vi "Select_Profile.vi"(0 "Enum":T1, 3 "error in":errorcluster) -> (7 "selected path":path, 10 "error out":errorcluster)   [LabVIEW 2021]
uses:
  test_type.ctl
  Template/Main_VI/Control/Ini.ctl
panel:
  out "All Files in Dir":path[](array[path])
  out "Array 2":path[](array[path])
  out "Ring - Menu 2":u16(ring) items=["acw_09June26_104916", "DCW_01June26_173303"]
  out "standard output":string
  in  "Back Button":bool
  in  "Select File":u16(ring) items=["ACW_15June26_202829", "DCW_01June26_173303", "DCW_16June26_152616", "IR-2_16June26_152710", "IR_15June26_203337", "IR_16June26_152633"]
  out "element":path
  out "filenames":string[](array[string])
  out "Array":string[](array[string])
  in  "Enum 2":T1
  in  "Select Button 2":bool
  out "selected path 2":path caption="selected path"
  in  "Select Button":bool
  # "PLEASE SELECT THE PROFILE"
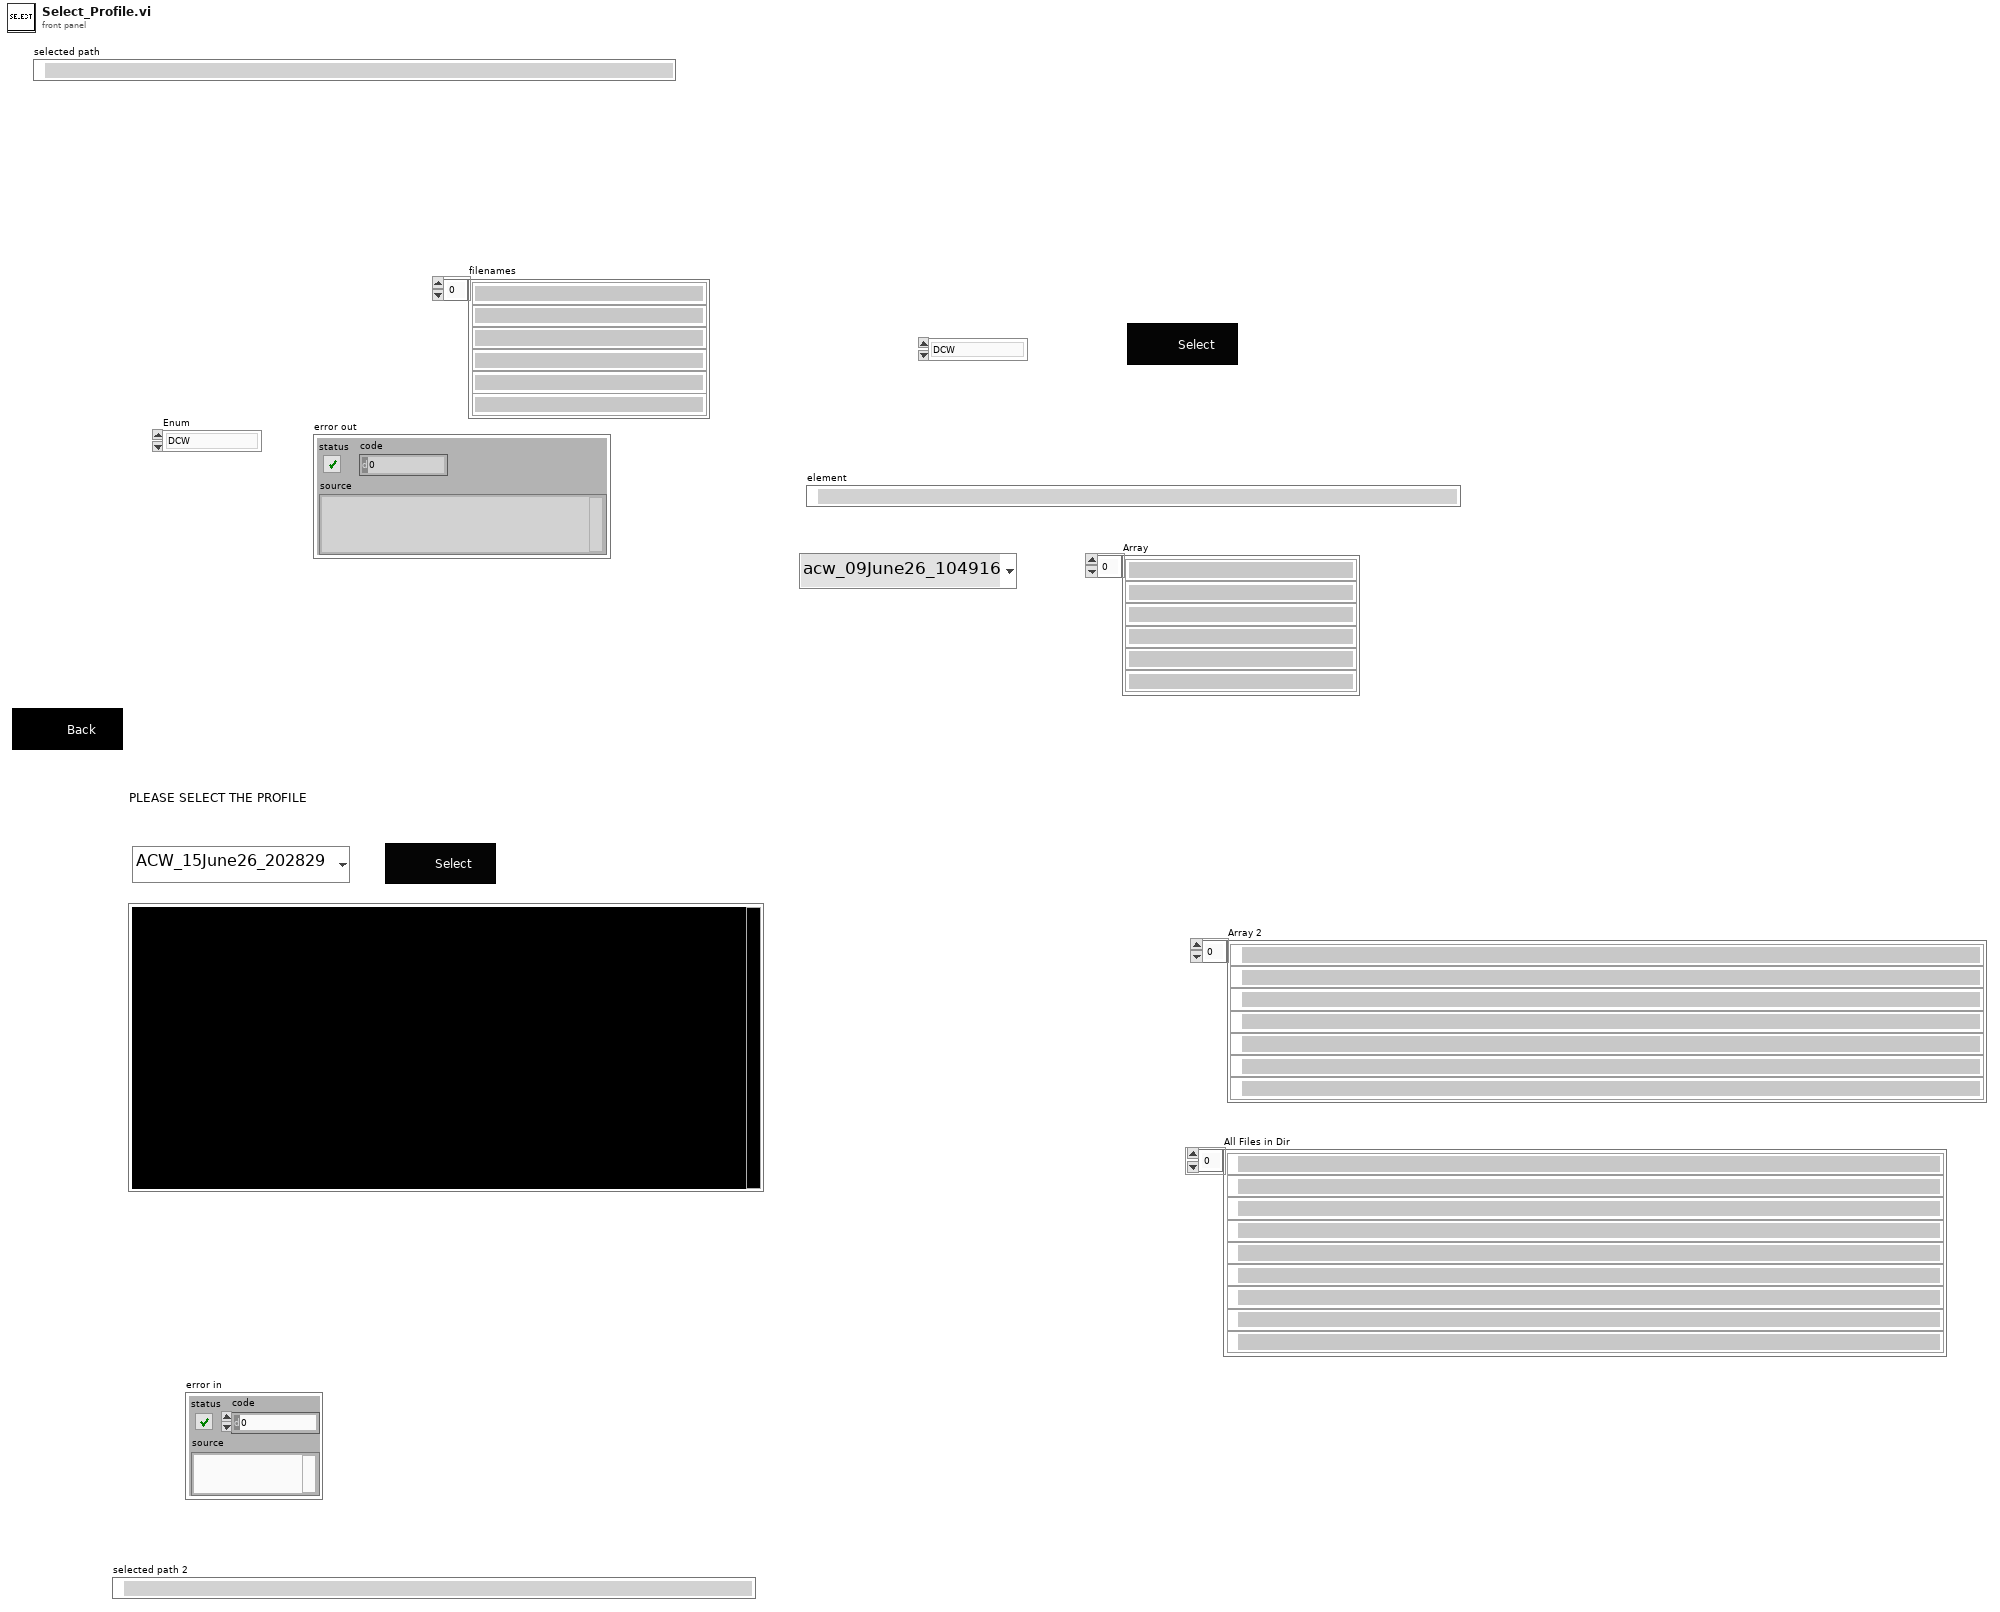
[diagram p1: front panel]
types:
  T1 = typedef "test_type.ctl" = enum16{"DCW", "ACW", "IR"}
  T2 = typedef "Ini.ctl" = enum16{"Write", "Read"}
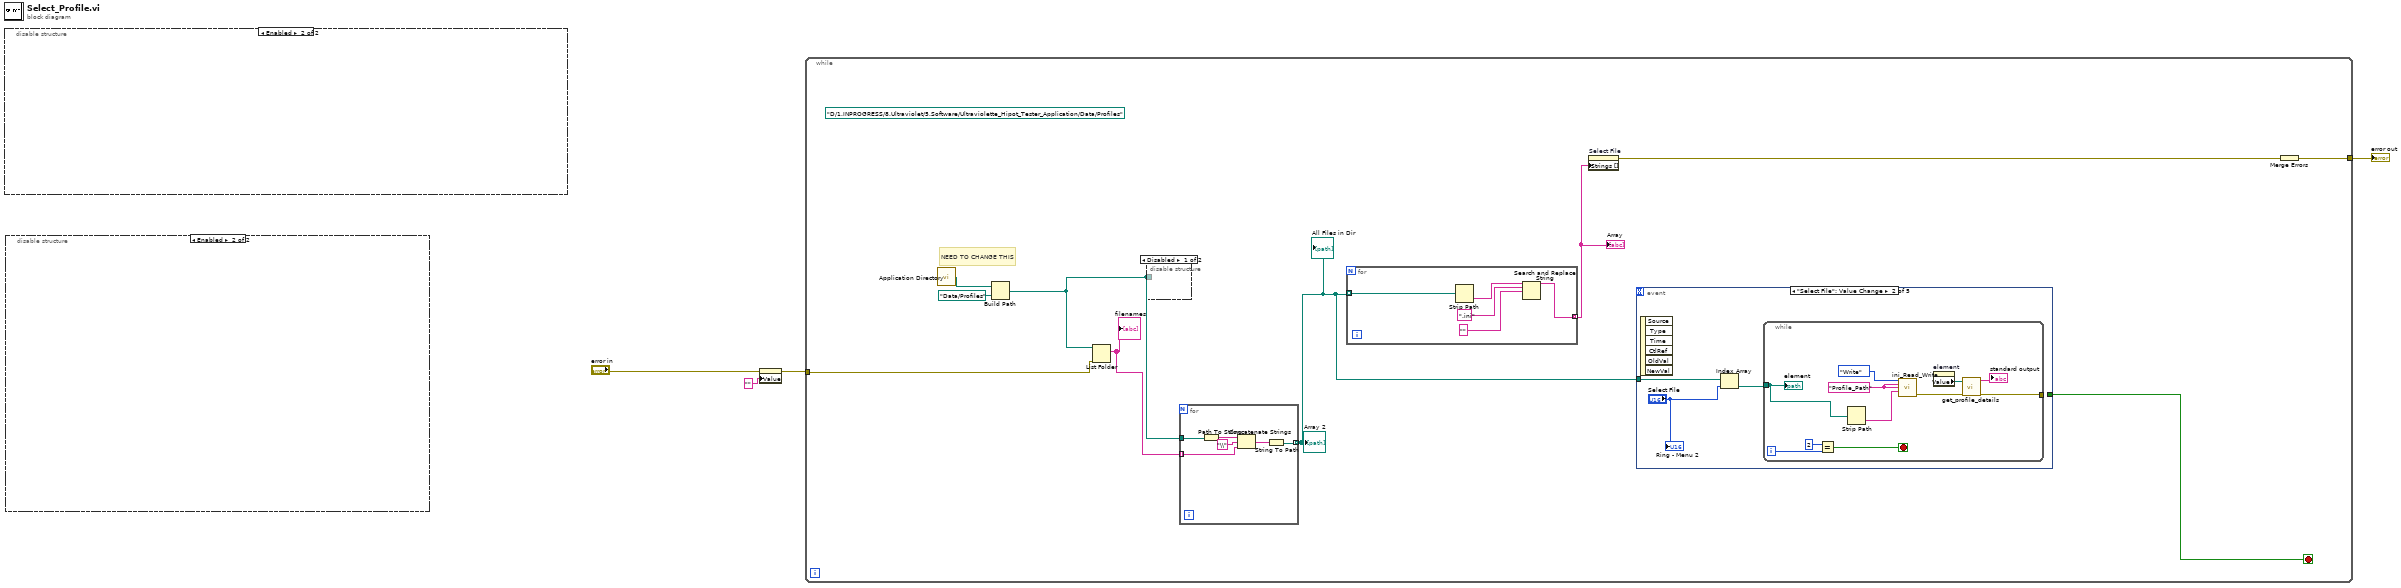
[diagram p0: block diagram]
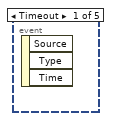
[diagram p3: hidden frame]
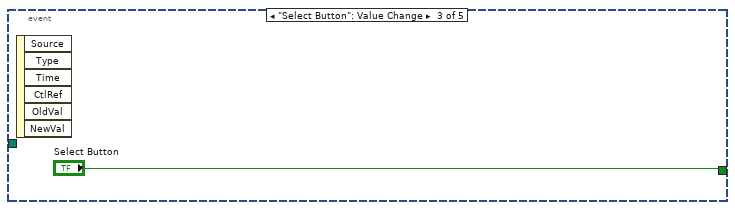
[diagram p4: hidden frame]
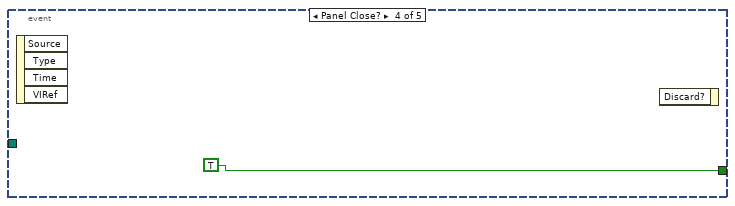
[diagram p5: hidden frame]
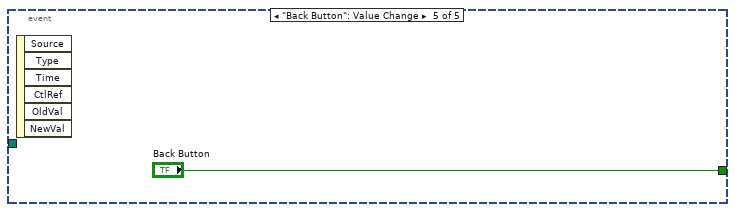
[diagram p6: hidden frame]
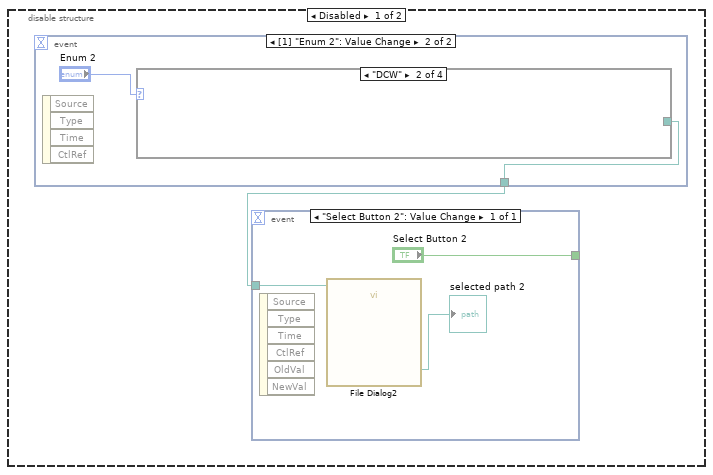
[diagram p7: hidden frame]
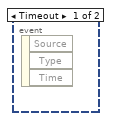
[diagram p8: hidden frame]
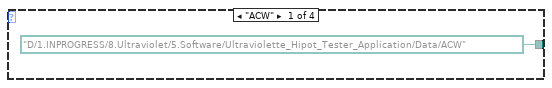
[diagram p9: hidden frame]
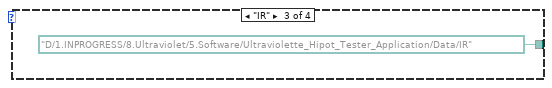
[diagram p10: hidden frame]
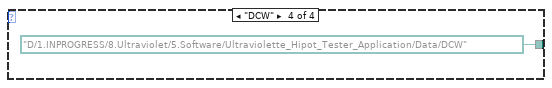
[diagram p11: hidden frame]
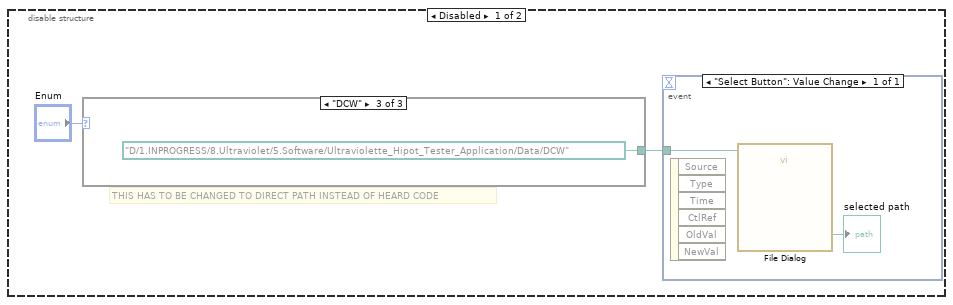
[diagram p12: hidden frame]
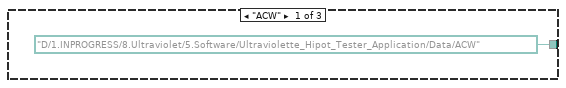
[diagram p13: hidden frame]
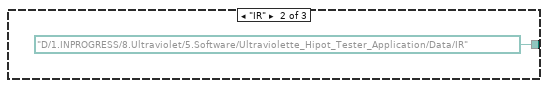
[diagram p14: hidden frame]
diagram:
  n1 = disable-structure shown="Enabled" {
    frame Disabled {
      # "THIS HAS TO BE CHANGED TO DIRECT PATH INSTEAD OF HEARD CODE"
      n2 = case shown="\"DCW\"" "Enum" {
        tunnel: [path "D:/1.INPROGRESS/8.Ultraviolet/5.Software/Ultraviolette_Hipot_Tester_Application/Data/ACW" ("start path") path "D:/1.INPROGRESS/8.Ultraviolet/5.Software/Ultraviolette_Hipot_Tester_Application/Data/IR" ("start path") path "D:/1.INPROGRESS/8.Ultraviolet/5.Software/Ultraviolette_Hipot_Tester_Application/Data/DCW" ("start path")] -> w5
        frame "ACW" {
        }
        frame "IR" {
        }
        frame "DCW" {
        }
      }
      n3 = event shown="[0] \"Select Button\": Value Change" {
        selector: _ -> [_]
        dyn-events: _ -> [_]
        timeout: _ -> [_]
        tunnel: w5 -> [w7]
        event "Select Button": Value Change {
          n4 = event-data() -> ()  [unwired: 1 in, 6 out]
          n5 = call "File Dialog"("start path"=w7) -> ("selected path"=→"selected path":path)  [unwired: 11 in, 3 out]
        }
      }
    }
    frame Enabled {
    }
  }
  n6 = disable-structure shown="Enabled" {
    frame Disabled {
      n7 = event shown="[1] \"Enum 2\": Value Change" {
        selector: _ -> [_ _]
        dyn-events: _ -> [_ _]
        timeout: _ -> [_ _]
        tunnel: [_ w14] -> w12
        event Timeout {
          n8 = event-data() -> ()  [unwired: 1 in, 3 out]
        }
        event Value Change {
          n9 = event-data() -> ()  [unwired: 1 in, 4 out]
          n10 = case shown="\"DCW\"" "Enum 2" {
            tunnel: [path "D:/1.INPROGRESS/8.Ultraviolet/5.Software/Ultraviolette_Hipot_Tester_Application/Data/ACW" ("start path") _ path "D:/1.INPROGRESS/8.Ultraviolet/5.Software/Ultraviolette_Hipot_Tester_Application/Data/IR" ("start path") path "D:/1.INPROGRESS/8.Ultraviolet/5.Software/Ultraviolette_Hipot_Tester_Application/Data/DCW" ("start path")] -> w14
            frame "ACW" {
            }
            frame "DCW" {
            }
            frame "IR" {
            }
            frame "DCW" {
            }
          }
        }
      }
      n11 = event shown="[0] \"Select Button 2\": Value Change" {
        selector: _ -> [_]
        dyn-events: _ -> [_]
        timeout: _ -> [_]
        tunnel: w12 -> [w20]
        tunnel: ["Select Button 2"] -> _
        event "Select Button 2": Value Change {
          n12 = event-data() -> ()  [unwired: 1 in, 6 out]
          n13 = call "File Dialog2"("start path"=w20) -> ("selected path"=→"selected path 2":path)  [unwired: 11 in, 3 out]
        }
      }
    }
    frame Enabled {
    }
  }
  n14 = property on="standard output" class="Str"(error in="error in", "Value"="" ("standard output")) -> (error out=w2:errorcluster)  [unwired: 1 in, 1 out]
  n15 = while {
    tunnel: [w28] -> w4
    tunnel: w2 -> [w27]
    stop <- w24 stop-if-true
    (unwired) path "D:/1.INPROGRESS/8.Ultraviolet/5.Software/Ultraviolette_Hipot_Tester_Application/Data/Profiles" ("start path")
    # "NEED TO CHANGE THIS"
    n16 = call <vilib>:"Application Directory.vi"() -> ("Application Directory"=w25:path)
    n17 = Build Path(base path=w25, name or relative path=path "Data/Profiles") -> (appended path=w21:path)
    n18 = List Folder(path=w21, error in=w27) -> (filenames=w23:string[])  [unwired: 2 in, 3 out]
    "filenames" <- w23
    n19 = disable-structure shown="Disabled" {
      disable-tunnel: w21 -> [w31 _]
      frame Disabled {
      }
      frame Enabled {
      }
    }
    n20 = for {
      tunnel: w21 -> [w37]
      tunnel: w23 -> [w34] mode=indexing
      tunnel: [w32] -> w22 mode=indexing
      n21 = Path To String(path=w37) -> (string=w36:string)
      n22 = Concatenate Strings(w36, "\\" ("string"), w34) -> (w33:string)
      n23 = String To Path(string=w33) -> (path=w32:path)
    }
    "Array 2" <- w22
    "All Files in Dir" <- w22
    n24 = for {
      tunnel: w22 -> [w59] mode=indexing
      tunnel: [w55] -> w30 mode=indexing
      n25 = Strip Path(path=w59) -> (name=w58:string)  [unwired: 1 out]
      n26 = Search and Replace String(input string=w58, search string=".ini", replace string="" ("replace string (\"\")")) -> (result string=w55:string)  [unwired: 5 in, 3 out]
    }
    "Array" <- w30
    n27 = property on="Select File" class="Ring (strict)"("Strings []"=w30) -> (error out=w29:errorcluster)  [unwired: 2 in, 1 out]
    n28 = event shown="[1] \"Select File\": Value Change" {
      selector: _ -> [_ _ _ _ _]
      dyn-events: _ -> [_ _ _ _ _]
      timeout: _ -> [_ _ _ _ _]
      tunnel: w22 -> [_ w40 _ _ _]
      tunnel: [_ _ "Select Button" TRUE "Back Button"] -> w24
      event Timeout {
        n29 = event-data() -> ()  [unwired: 1 in, 3 out]
      }
      event "Select File": Value Change {
        n30 = event-data() -> ()  [unwired: 1 in, 6 out]
        n31 = Index Array(array=w40, index="Select File") -> (element=w39:path)
        n32 = while {
          tunnel: [w47] -> _
          tunnel: w39 -> [w42]
          i -> [w46]
          stop <- w45 stop-if-true
          w50 = "Profile_Path" ("Read Section")
          n33 = Equal?(x=2, y=w46) -> (x = y?=w45:bool)
          n34 = Strip Path(path=w42) -> (name=w41:string)  [unwired: 1 out]
          n35 = call "ini_Read_Write.vi"(0:Ini."Write", "Write Section"=w50, "Write key"=w50, "Write"=w41) -> ("error in (no error) 3"=w48:errorcluster)  [unwired: 10 in, 1 out]
          n36 = property on="element" class="Path"() -> ("Value"=w49:path)  [unwired: 2 in, 2 out]
          n37 = call "get_profile_details.vi"("error in (no error)"=w48, "path"=w49) -> ("error out"=w47:errorcluster, "standard output"=→"standard output":string)  [unwired: 8 in]
          "element" <- w42
        }
        "Ring - Menu 2" <- "Select File"
      }
      event "Select Button": Value Change {
        n38 = event-data() -> ()  [unwired: 1 in, 6 out]
      }
      event Panel Close? {
        n39 = event-data() -> ()  [unwired: 1 in, 4 out]
        n40 = event-data() -> ()  [unwired: 2 in, 1 out]
      }
      event "Back Button": Value Change {
        n41 = event-data() -> ()  [unwired: 1 in, 6 out]
      }
    }
    n42 = Merge Errors(w29) -> (w28:errorcluster)
  }
  "error out" <- w4
